vi "TDR Feature.vi"(9 ".pinmap File Path":path, 11 "TDR File Path":path) -> (1 "spreadsheet string":string, 3 "Offset Delay":dbl[](array[numeric]))   [LabVIEW 2025, in "Digital Pattern Sequencer.lvclass"]
uses:
  Digital Pattern Sequencer.lvclass
  Digital Pattern Sequencer.lvclass/Digital Pattern Sequencer.ctl
  <resource>/objmgr/DOMUserDefRef.rc
  <vilib>/xml/NI_XML.lvlib
  <vilib>/xml/Load XML String.vi
  <vilib>/xml/XPath/Get All Matched Nodes (String).vi
panel:
  out "Pin Name":string[](array[string])
  out "Channel Number":string[](array[string])
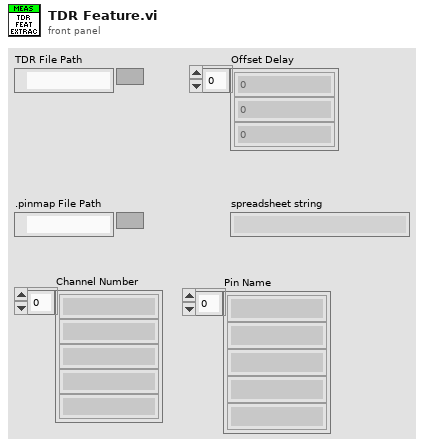
[diagram p1: front panel]
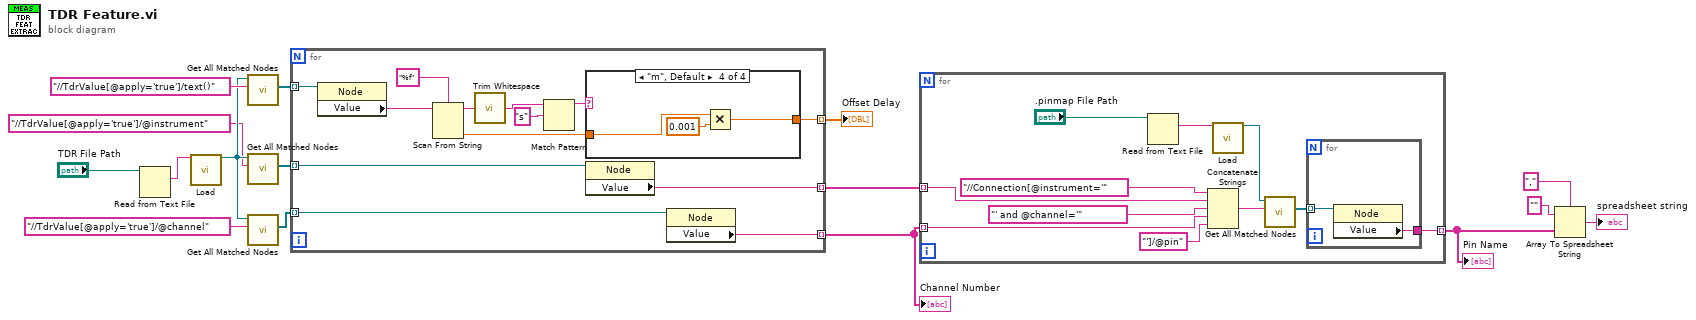
[diagram p0: block diagram]
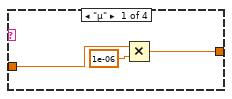
[diagram p2: hidden frame]
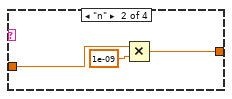
[diagram p3: hidden frame]
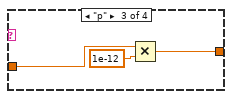
[diagram p4: hidden frame]
diagram:
  n1 = Read from Text File(file (use dialog)="TDR File Path") -> (text=w15:string)  [unwired: 3 in, 3 out]
  n2 = call-poly <vilib>:"Load.vi"("XML string"=w15) -> ("DOM document out"=w9:refnum<k20>)  [unwired: 12 in, 2 out]
  n3 = call-poly <vilib>:"Get All Matched Nodes.vi"("XPath expression"="//TdrValue[@apply='true']/text()", "node in"=w9) -> ("node result array"=w16:refnum<k20>[])  [unwired: 7 in, 2 out]
  n4 = call-poly <vilib>:"Get All Matched Nodes.vi"("XPath expression"="//TdrValue[@apply='true']/@instrument", "node in"=w9) -> ("node result array"=w7:refnum<k20>[])  [unwired: 7 in, 2 out]
  n5 = call-poly <vilib>:"Get All Matched Nodes.vi"("XPath expression"="//TdrValue[@apply='true']/@channel", "node in"=w9) -> ("node result array"=w11:refnum<k20>[])  [unwired: 7 in, 2 out]
  n6 = for {
    tunnel: w16 -> [w29] mode=indexing
    tunnel: [w20] -> w5 mode=indexing
    tunnel: w11 -> [w28] mode=indexing
    tunnel: [w27] -> w10 mode=indexing
    tunnel: w7 -> [w26] mode=indexing
    tunnel: [w25] -> w6 mode=indexing
    n7 = property class="Node"(reference=w29) -> ("Value"=w24:string)  [unwired: 1 in, 2 out]
    n8 = Scan From String(format string="%f", input string=w24) -> (remaining string=w17:string, output 1=w19:dbl)  [unwired: 3 in, 2 out]
    n9 = call-poly <vilib>:"Trim Whitespace.vi"("string"=w17) -> ("trimmed string"=w18:string)  [unwired: 1 in]
    n10 = Match Pattern(string=w18, regular expression="s") -> (before substring=w21:string)  [unwired: 1 in, 3 out]
    n11 = case shown="\"m\", Default" w21 {
      tunnel: w19 -> [w31 w34 w37 w41]
      tunnel: [w30 w33 w36 w39] -> w20
      frame "µ" {
        n12 = Multiply(x=w31, y=1e-06) -> (x*y=w30:dbl)
      }
      frame "n" {
        n13 = Multiply(x=w34, y=1e-09) -> (x*y=w33:dbl)
      }
      frame "p" {
        n14 = Multiply(x=w37, y=1e-12) -> (x*y=w36:dbl)
      }
      frame "m", Default {
        n15 = Multiply(x=w41, y=0.001) -> (x*y=w39:dbl)
      }
    }
    n16 = property class="Node"(reference=w26) -> ("Value"=w25:string)  [unwired: 1 in, 2 out]
    n17 = property class="Node"(reference=w28) -> ("Value"=w27:string)  [unwired: 1 in, 2 out]
  }
  "Channel Number" <- w10
  "Offset Delay" <- w5
  n18 = for {
    tunnel: w10 -> [w43] mode=indexing
    tunnel: [w45] -> w4 mode=indexing
    tunnel: w6 -> [w44] mode=indexing
    n19 = Read from Text File(file (use dialog)=".pinmap File Path") -> (text=w50:string)  [unwired: 3 in, 3 out]
    n20 = Concatenate Strings("//Connection[@instrument='" ("string"), w44, "' and @channel='" ("string"), w43, "']/@pin" ("string")) -> (w47:string)
    n21 = call-poly <vilib>:"Load.vi"("XML string"=w50) -> ("DOM document out"=w51:refnum<k20>)  [unwired: 12 in, 2 out]
    n22 = call-poly <vilib>:"Get All Matched Nodes.vi"("XPath expression"=w47, "node in"=w51) -> ("node result array"=w52:refnum<k20>[])  [unwired: 7 in, 2 out]
    n23 = for {
      tunnel: w52 -> [w54] mode=indexing
      tunnel: [w53] -> w45
      n24 = property class="Node"(reference=w54) -> ("Value"=w53:string)  [unwired: 1 in, 2 out]
    }
  }
  "Pin Name" <- w4
  n25 = Array To Spreadsheet String(delimiter (Tab)=",", array=w4, 3:"" ("format string")) -> (spreadsheet string=→"spreadsheet string":string)
